vi "WriteToDictionary.vi"(6 "Initial call":bool, 7 "Section":string[](array[string]), 8 "error in (no error)":errorcluster, 9 "Content":T1[](array[typedef]), 10 "Keys":string[](array[string]), 11 "ConfigManager.Text in":refnum<class "ConfigManager.Text.lvclass">) -> (0 "error out":errorcluster, 3 "ConfigManager.Text out":refnum<class "ConfigManager.Text.lvclass">)   [LabVIEW 2013, in "CfgManager.Text.lvlib" / "ConfigManager.Text.lvclass"]
uses:
  ConfigManager.Text.lvclass
  Dictionary Payload -- cluster.ctl
  ConfigManager.Text.lvclass/ConfigManager.Text.ctl
  <vilib>/Utility/error.llb/Clear Errors.vi
  <vilib>/LabVIEW Open Source Project/Unicity/Delimiter/Delimiter.lvclass
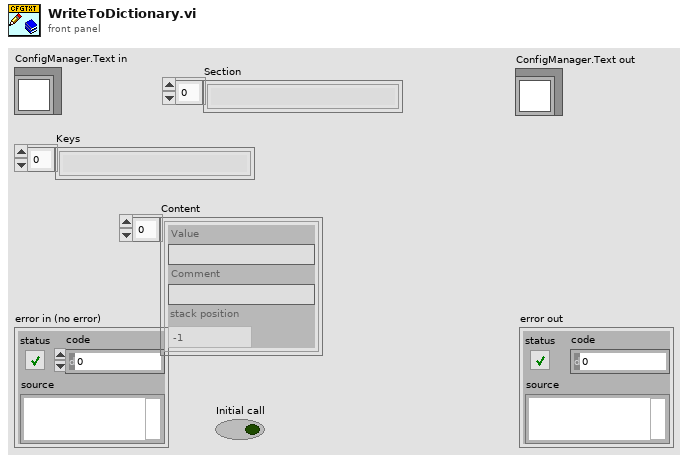
[diagram p1: front panel]
types:
  T1 = typedef "CfgManager.Text.lvlib/ConfigManager.Text.lvclass/Dictionary Payload -- cluster.ctl" = cluster{"Value":string, "Comment":string, "stack position":i32}
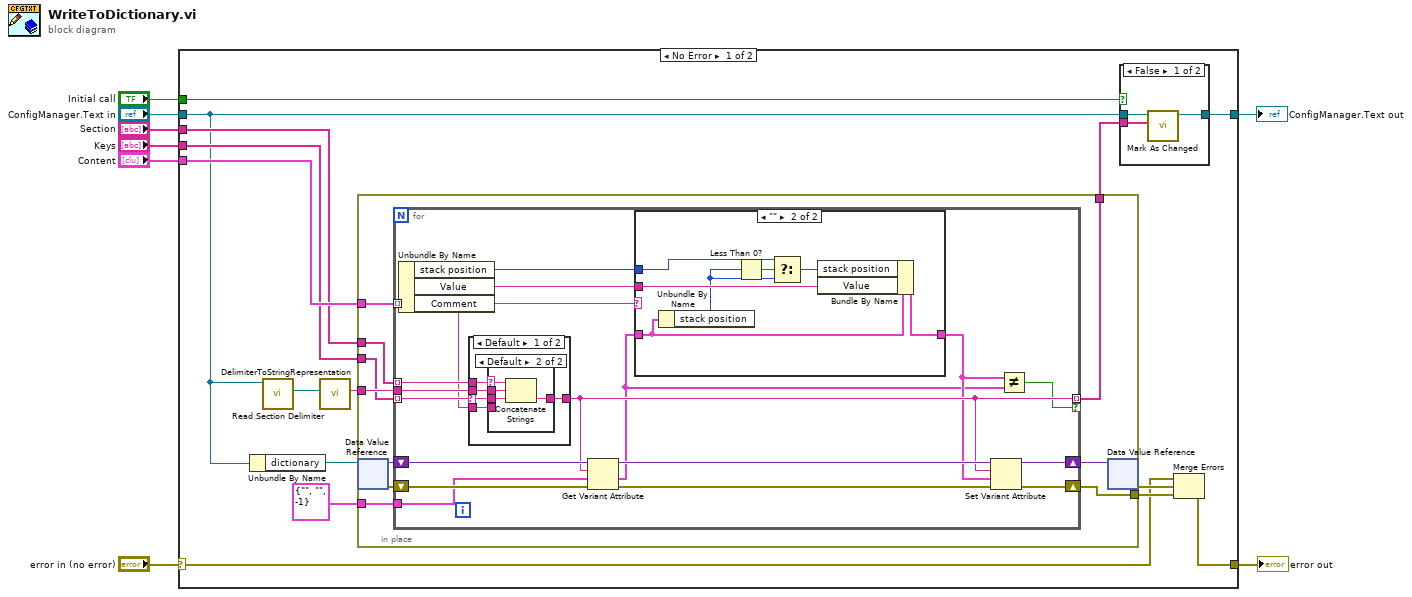
[diagram p0: block diagram]
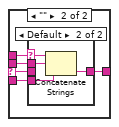
[diagram p4: hidden frame]
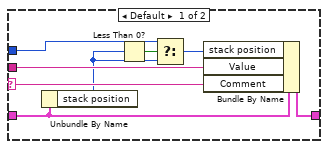
[diagram p6: hidden frame]
diagram:
  n1 = case shown="No Error" "error in (no error)" {
    selector: "error in (no error)" -> [w18 w92]
    tunnel: [w23 w92] -> w8
    tunnel: "Content" -> [w20 _]
    tunnel: "Keys" -> [w17 _]
    tunnel: "ConfigManager.Text in" -> [w12 w91]
    tunnel: [w14 w91] -> w3
    tunnel: "Section" -> [w16 _]
    tunnel: "Initial call" -> [w10 _]
    frame No Error {
      n2 = Unbundle By Name(w12) -> ("dictionary"=w19:refnum<data-value>)
      n3 = call "Read Section Delimiter.vi"("ConfigManager.Text in"=w12) -> ("Section Delimiter"=w11:refnum<class "Delimiter.lvclass">)  [unwired: 9 in, 1 out]
      n4 = call <vilib>:"DelimiterToStringRepresentation.vi"("Delimiter"=w11) -> ("String representation"=w15:string)  [unwired: 10 in]
      n5 = in-place {
        in-place-border: w17 -> [w29]
        in-place-border: w20 -> [w30]
        in-place-border: [w34] -> w22
        in-place-border: w16 -> [w28]
        in-place-border: w15 -> [w32]
        in-place-border: [w33] -> w13
        in-place-border: T1 {"Value"="", "Comment"="", "stack position"=-1} ("Dictionary Payload") -> [w31]
        n6 = in-place-dvr #1(w19) -> (w37:variant, w35:errorcluster)
        n7 = for {
          shift-right: [w55] -> w36
          shift-left: w37 -> [w51]
          tunnel: w29 -> [w41] mode=indexing
          tunnel: w30 -> [w45] mode=indexing
          shift-right: [w54] -> w34
          shift-left: w35 -> [w49]
          tunnel: w28 -> [w53] mode=indexing
          tunnel: w32 -> [w52]
          tunnel: [w46] -> w33 mode=indexing if=w42
          tunnel: w31 -> [w47]
          n8 = Unbundle By Name(w45) -> ("stack position"=w39:i32, "Value"=w44:string, "Comment"=w40:string)
          n9 = case shown="Default" w41 {
            selector: w41 -> [w57 w67]
            tunnel: w53 -> [w60 w70]
            tunnel: w52 -> [w59 w69]
            tunnel: [w58 w68] -> w46
            tunnel: w40 -> [w56 w66]
            frame Default {
              n10 = case shown="Default" w60 {
                selector: w60 -> [_ w62]
                tunnel: w57 -> [w61 w65]
                tunnel: [w61 w64] -> w58
                tunnel: w59 -> [_ w63]
                tunnel: w56 -> [_ _]
                frame "" {
                }
                frame Default {
                  n11 = Concatenate Strings(w62, w63, w65) -> (w64:string)
                }
              }
            }
            frame "" {
              n12 = case shown="Default" w70 {
                selector: w70 -> [_ w73]
                tunnel: w67 -> [_ _]
                tunnel: [w71 w75] -> w68
                tunnel: w69 -> [_ w74]
                tunnel: w66 -> [w71 w72]
                frame "" {
                }
                frame Default {
                  n13 = Concatenate Strings(w73, w74, w72) -> (w75:string)
                }
              }
            }
          }
          n14 = Get Variant Attribute(Variant=w51, name=w46, default value (empty Variant)=w47, error in=w49) -> (duplicate Variant=w50:variant, value=w38:T1, error out=w48:errorcluster)  [unwired: 1 out]
          n15 = case shown="\"\"" w40 {
            selector: w40 -> [w82 _]
            tunnel: [w81 w89] -> w43
            tunnel: w38 -> [w80 w84]
            tunnel: w44 -> [w83 w90]
            tunnel: w39 -> [w77 w86]
            frame Default {
              n16 = Unbundle By Name(w80) -> ("stack position"=w78:i32)
              n17 = Less Than 0?(x=w78) -> (x < 0?=w79:bool)
              n18 = Select(t=w77, s=w79, f=w78) -> (s? t:f=w76:i32)
              n19 = Bundle By Name(cluster=w80, "stack position"=w76, "Value"=w83, "Comment"=w82) -> (w81:T1)
            }
            frame "" {
              n20 = Unbundle By Name(w84) -> ("stack position"=w87:i32)
              n21 = Less Than 0?(x=w87) -> (x < 0?=w88:bool)
              n22 = Select(t=w86, s=w88, f=w87) -> (s? t:f=w85:i32)
              n23 = Bundle By Name(cluster=w84, "stack position"=w85, "Value"=w90) -> (w89:T1)
            }
          }
          n24 = Set Variant Attribute(Variant=w50, name=w46, value=w43, error in=w48) -> (Variant out=w55:variant, error out=w54:errorcluster)  [unwired: 1 out]
          n25 = Not Equal?(x=w43, y=w38) -> (x != y?=w42:bool)
        }
        n26 = in-place-dvr #1(w36) -> (w21:errorcluster)  [unwired: 1 out]
      }
      n27 = case shown="False" w10 {
        tunnel: [w26 w27] -> w14
        tunnel: w13 -> [w25 _]
        tunnel: w12 -> [w24 w27]
        frame False {
          n28 = call "Mark As Changed.vi"("Changed elements"=w25, "ConfigManager.Text in"=w24) -> ("ConfigManager.Text out"=w26:refnum<class "ConfigManager.Text.lvclass">)  [unwired: 9 in]
        }
        frame True {
        }
      }
      n29 = Merge Errors(w18, w21, w22) -> (w23:errorcluster)
    }
    frame Error {
    }
  }
  "error out" <- w8
  "ConfigManager.Text out" <- w3
